vi "DAQmx Test.vi"   [LabVIEW 2020, in "VolatusScratch.lvlib"]
uses:
  VolatusScratch.lvlib
  Volatus/Volatus Core/Volatus Core.lvclass
  VolatusDAQ/VolatusDAQ.lvlib
  VolatusDAQGenericGUI/VolatusDAQGenericGUI.lvlib
  VolatusData/VolatusData.lvlib
panel:
  # "DAQmx Test App"
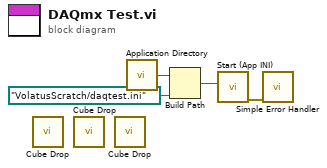
[diagram p0: block diagram]
diagram:
  n1 = call "Cube Drop.vi"() -> ()  [unwired: 12 in]
  n2 = call "Cube Drop.vi"() -> ()  [unwired: 12 in]
  n3 = call "Cube Drop.vi"() -> ()  [unwired: 12 in]
  n4 = call <vilib>:"Application Directory.vi"() -> ("Application Directory"=w3:path)
  n5 = Build Path(base path=w3, name or relative path=path "VolatusScratch/daqtest.ini") -> (appended path=w1:path)
  n6 = call "Start (App INI).vi"("INI Path (Default)"=w1) -> ("error out"=w4:errorcluster)  [unwired: 9 in, 1 out]
  n7 = call <vilib>:"Simple Error Handler.vi"("error in (no error)"=w4) -> ()  [unwired: 4 in, 5 out]
